vi "calculator.vi"() -> ()   [LabVIEW 2025]
uses:
  <vilib>/ErrorRing/Error Ring.xnode
panel:
  out "Run Time":string
  out "History":string[](array[string])
  out "result":dbl
  out "result str":string
  out "`()` count":u16
  in  "1/x":bool
  out "input queue":cluster{"op":u16, "number":dbl}[](array[cluster])
  in  "Stop":bool
  out "Current Time":string
  in  "C":bool
  in  "CE":bool
  in  "backspace":bool
  in  "sqrt":bool
  in  "+/-":bool
  in  "/":bool
  in  "=":bool
  in  "*":bool
  in  "-":bool
  in  "+":bool
  in  ".":bool
  in  "0":bool
  in  ")":bool
  in  "(":bool
  in  "9":bool
  in  "8":bool
  in  "7":bool
  in  "6":bool
  in  "5":bool
  in  "4":bool
  in  "3":bool
  in  "2":bool
  in  "1":bool
  out "screen":string
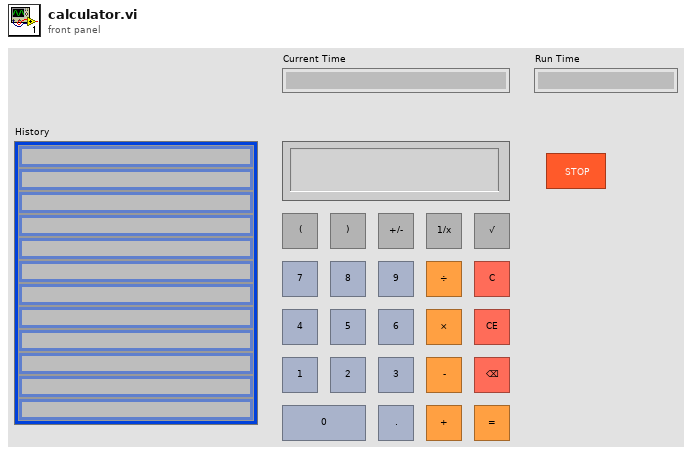
[diagram p1: front panel]
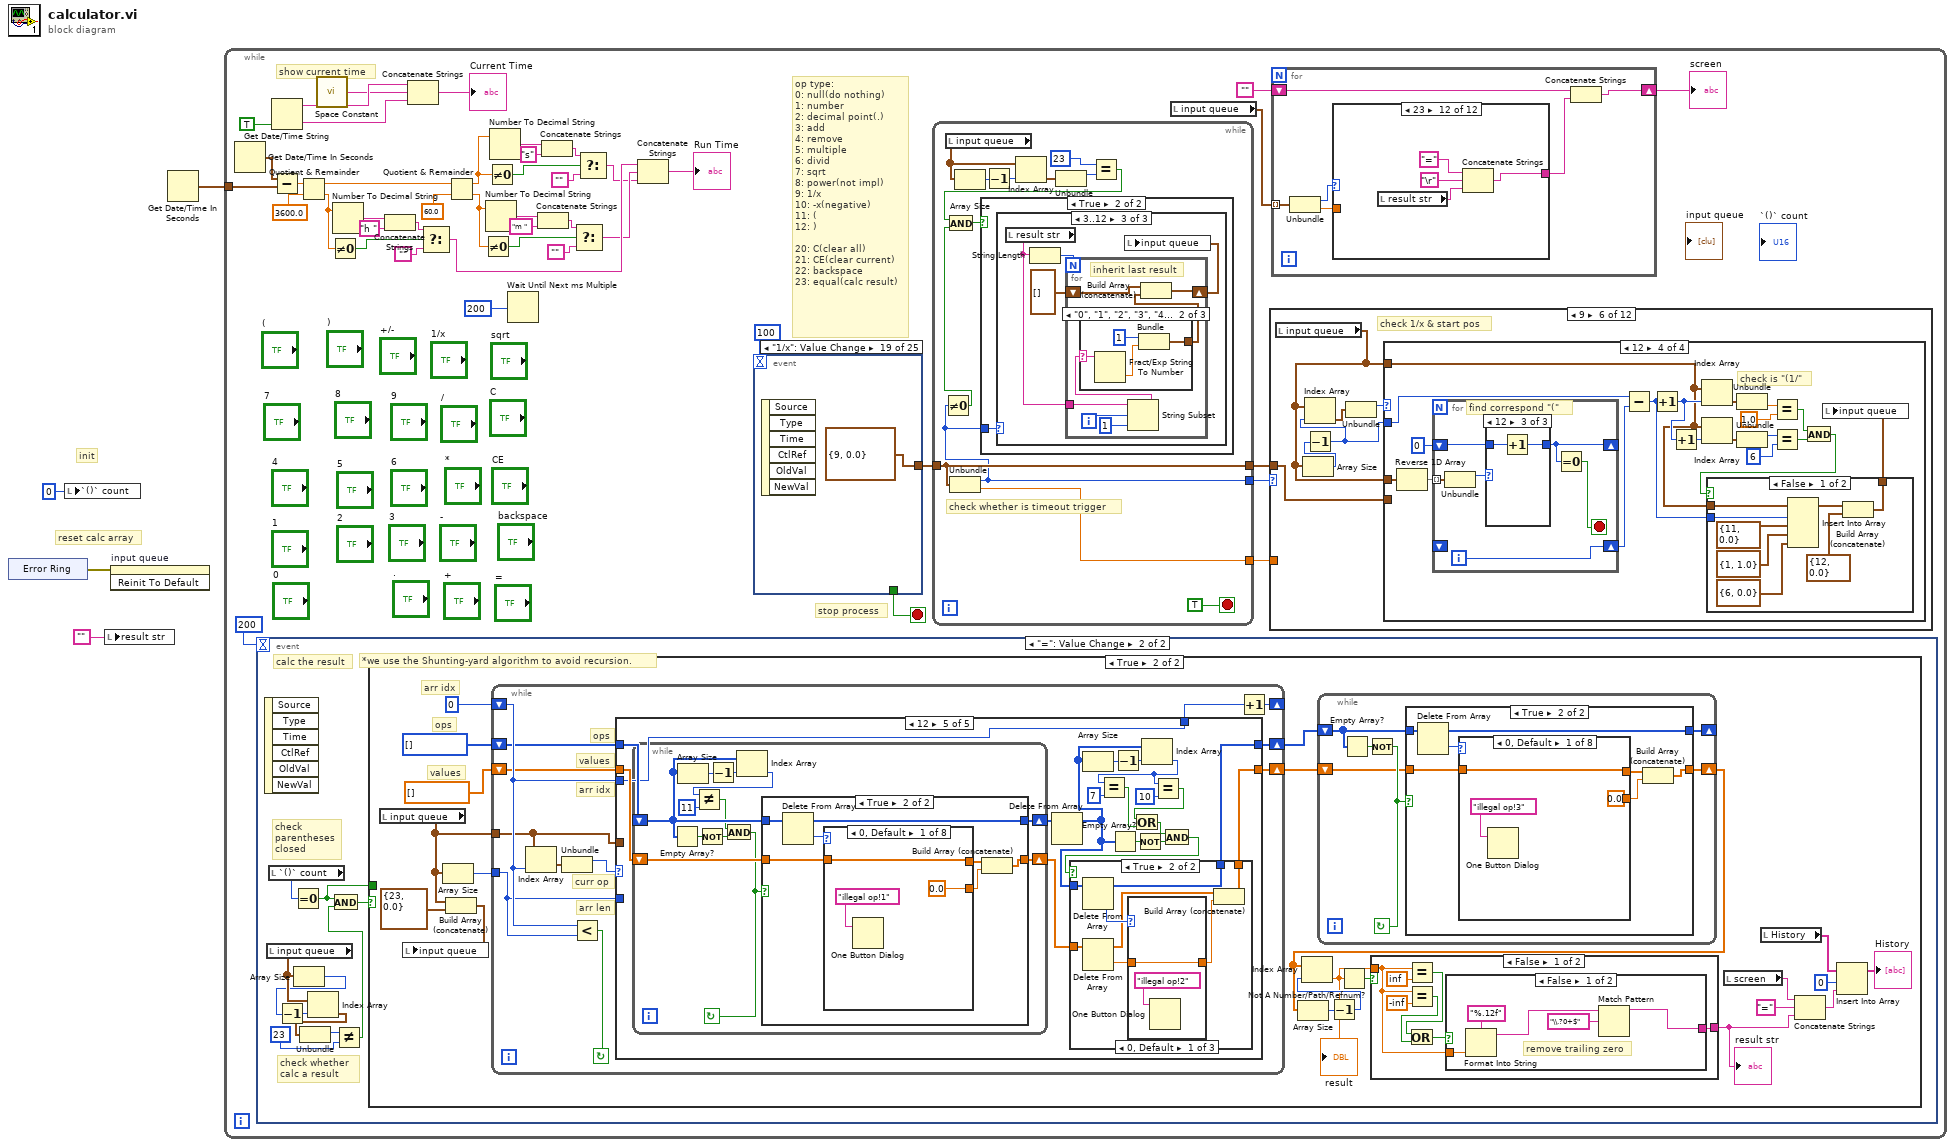
[diagram p0: block diagram]
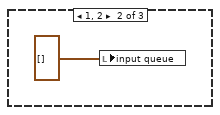
[diagram p4: hidden frame]
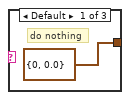
[diagram p5: hidden frame]
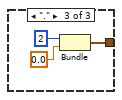
[diagram p6: hidden frame]
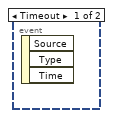
[diagram p7: hidden frame]
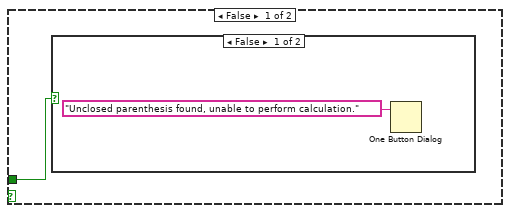
[diagram p8: hidden frame]
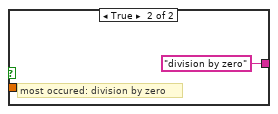
[diagram p10: hidden frame]
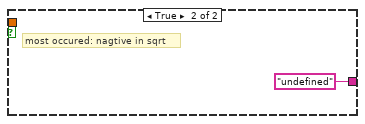
[diagram p11: hidden frame]
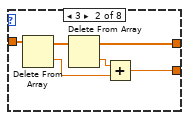
[diagram p13: hidden frame]
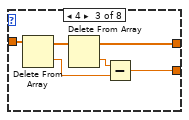
[diagram p14: hidden frame]
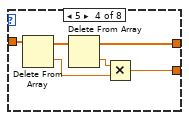
[diagram p15: hidden frame]
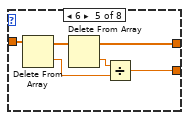
[diagram p16: hidden frame]
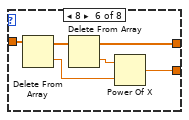
[diagram p17: hidden frame]
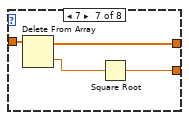
[diagram p18: hidden frame]
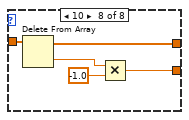
[diagram p19: hidden frame]
diagram:
  # "init"
  # "reset calc array"
  n1 = xnode "Error Ring"() -> ("error out"=w4:errorcluster)
  n2 = local write "`()` count"(u16 0 ("`()` count")) -> ()
  n3 = local write "result str"("" ("result str")) -> ()
  n4 = invoke on="input queue" class="Arr (strict)" method="Reinit To Default"(error in=w4) -> ()  [unwired: 2 in, 3 out]
  n5 = Get Date/Time In Seconds() -> (seconds since 1Jan1904=w1:timestamp)
  n6 = while {
    tunnel: w1 -> [w32]
    stop <- w37 stop-if-true
    # "stop process"
    # "op type:\n0: null(do nothing)\n1: number\n2: decimal point(.)\n3: add\n4: remove\n5: multiple\n6: divid\n7: sqrt\n8: power(not impl)\n9: 1/x\n10: -x(negative)\n11: (\n12: )\n\n20: C(clear all)\n21: CE(clear current)\n22: backspace\n23: equal(calc result)"
    # "show current time"
    n7 = Get Date/Time In Seconds() -> (seconds since 1Jan1904=w31:timestamp)
    n8 = event shown="[1] \"=\": Value Change" {
      selector: _ -> [_ _]
      dyn-events: _ -> [_ _]
      timeout: 200 -> [_ _]
      event Timeout {
        n9 = event-data() -> ()  [unwired: 1 in, 3 out]
      }
      event "=": Value Change {
        # "check whether\ncalc a result"
        # "check\nparentheses\nclosed"
        # "*we use the Shunting-yard algorithm to avoid recursion."
        # "calc the result"
        n10 = event-data() -> ()  [unwired: 1 in, 6 out]
        n11 = local read "input queue"() -> (w89:cluster{"op":u16, "number":dbl}[])
        n12 = local read "`()` count"() -> (w92:u16)
        n13 = Equal To 0?(x=w92) -> (x = 0?=w83:bool)
        n14 = Array Size(array=w89) -> (size(s)=w87:i32)
        n15 = Decrement(x=w87) -> (x-1=w88:i32)
        n16 = Index Array(array=w89, index=w88) -> (element=w90:cluster{"op":u16, "number":dbl})
        n17 = Unbundle(w90) -> ("op"=w91:u16)  [unwired: 1 out]
        n18 = Not Equal?(x=w91, y=u16 23) -> (x != y?=w85:bool)
        n19 = And(x=w83, y=w85) -> (x .and. y?=w84:bool)
        n20 = case shown="True" w84 {
          tunnel: w83 -> [w93 _]
          frame False {
            n21 = case shown="False" w93 {
              frame False {
                n22 = One Button Dialog(message="Unclosed parenthesis found, unable to perform calculation.") -> ()  [unwired: 1 in, 1 out]
              }
              frame True {
              }
            }
          }
          frame True {
            # "arr idx"
            # "ops"
            # "values"
            n23 = local read "input queue"() -> (w97:cluster{"op":u16, "number":dbl}[])
            n24 = Array Size(array=w97) -> (size(s)=w98:i32)
            n25 = Build Array (concatenate)(w97, cluster{u16, dbl} {23, 0.0}) -> (w96:cluster{"op":u16, "number":dbl}[])
            n26 = local write "input queue"(w96) -> ()
            n27 = while {
              shift-right: [w187] -> w111
              shift-left: dbl[] [] -> [w192]
              shift-right: [w194] -> w112
              shift-left: u16[] [] -> [w193]
              shift-right: [w190] -> _
              shift-left: 0 -> [w195]
              tunnel: w98 -> [w188]
              tunnel: w97 -> [w189]
              stop <- w198 continue-if-true
              # "values"
              # "ops"
              # "arr idx"
              # "arr len"
              # "curr op"
              n28 = Index Array(array=w189, index=w195) -> (element=w197:cluster{"op":u16, "number":dbl})
              n29 = Unbundle(w197) -> ("op"=w196:u16)  [unwired: 1 out]
              n30 = Less?(x=w195, y=w188) -> (x < y?=w198:bool)
              n31 = case shown="12" w196 {
                selector: w196 -> [_ _ w255 w317 _]
                tunnel: w195 -> [_ w215 w256 w319 w330]
                tunnel: [w200 w214 w256 w319 w330] -> w191
                tunnel: w188 -> [w200 w213 _ _ _]
                tunnel: [w201 w204 w254 w316 w320] -> w194
                tunnel: w193 -> [w201 w203 w253 w318 w338]
                tunnel: [w199 w209 w250 w315 w321] -> w187
                tunnel: w192 -> [w199 w210 w252 w315 w337]
                tunnel: w189 -> [_ w212 _ _ _]
                frame 0, Default {
                }
                frame 1 {
                  n32 = while {
                    shift-right: [w230] -> w211
                    shift-left: "" -> [w231]
                    shift-right: [w224] -> w214
                    shift-left: w215 -> [w225]
                    tunnel: w213 -> [w236]
                    tunnel: w212 -> [w235]
                    stop <- w226 continue-if-true
                    n33 = Index Array(array=w235, index=w225) -> (element=w234:cluster{"op":u16, "number":dbl})
                    n34 = Unbundle(w234) -> ("op"=w233:u16, "number"=w232:dbl)
                    n35 = Less?(x=w225, y=w236) -> (x < y?=w228:bool)
                    n36 = case shown="2" w233 {
                      tunnel: w232 -> [_ w245 _]
                      tunnel: ["" w244 "."] -> w229
                      tunnel: [FALSE TRUE TRUE] -> w227
                      tunnel: w225 -> [w238 w242 w246]
                      tunnel: [w237 w241 w247] -> w224
                      frame 0, Default {
                        n37 = Decrement(x=w238) -> (x-1=w237:i32)
                      }
                      frame 1 {
                        n38 = Number To Decimal String(number=w245) -> (decimal integer string=w244:string)  [unwired: 1 in]
                        n39 = Increment(x=w242) -> (x+1=w241:i32)
                      }
                      frame 2 {
                        n40 = Increment(x=w246) -> (x+1=w247:i32)
                      }
                    }
                    n41 = And(x=w227, y=w228) -> (x .and. y?=w226:bool)
                    n42 = Concatenate Strings(w231, w229) -> (w230:string)
                  }
                  n43 = Fract/Exp String To Number(string=w211) -> (number=w206:dbl)  [unwired: 3 in, 1 out]
                  n44 = Array Size(array=w203) -> (size(s)=w208:i32)
                  n45 = Decrement(x=w208) -> (x-1=w202:i32)
                  n46 = Index Array(array=w203, index=w202) -> (element=w207:u16)
                  n47 = case shown="10" w207 {
                    tunnel: w206 -> [w218 w223]
                    tunnel: [w218 w221] -> w205
                    tunnel: w203 -> [w217 w220]
                    tunnel: [w217 w219] -> w204
                    frame 0, Default {
                    }
                    frame 10 {
                      n48 = Delete From Array(array=w220) -> (array with subset deleted=w219:u16[])  [unwired: 2 in, 1 out]
                      n49 = Multiply(x=w223, y=-1.0) -> (x*y=w221:dbl)
                    }
                  }
                  n50 = Build Array (concatenate)(w210, w205) -> (w209:dbl[])
                }
                frame 3..6 {
                  n51 = while {
                    tunnel: w255 -> [w264]
                    shift-right: [w257] -> w250
                    shift-left: w252 -> [w259]
                    shift-right: [w258] -> w251
                    shift-left: w253 -> [w260]
                    stop <- w261 continue-if-true
                    n52 = case shown="3, 4" w264 {
                      tunnel: [i16 0 i16 1 i16 2 i16 3] -> w263
                      frame 0, Default {
                      }
                      frame 3, 4 {
                      }
                      frame 5, 6 {
                      }
                      frame 7 {
                      }
                    }
                    n53 = Empty Array?(array=w260) -> (empty?=w277:bool)
                    n54 = Array Size(array=w260) -> (size(s)=w275:i32)
                    n55 = Decrement(x=w275) -> (x-1=w274:i32)
                    n56 = Not(x=w277) -> (.not. x?=w276:bool)
                    n57 = Index Array(array=w260, index=w274) -> (element=w266:u16)
                    n58 = Not Equal?(x=w266, y=u16 7) -> (x != y?=w269:bool)
                    n59 = Not Equal?(x=w266, y=u16 11) -> (x != y?=w267:bool)
                    n60 = Not Equal?(x=w266, y=u16 12) -> (x != y?=w268:bool)
                    n61 = case shown="3, 4" w266 {
                      tunnel: [i16 0 i16 1 i16 2 i16 3] -> w265
                      frame 0, Default {
                      }
                      frame 3, 4 {
                      }
                      frame 5, 6 {
                      }
                      frame 7 {
                      }
                    }
                    n62 = Compound Arithmetic op=AND(w269, w267, w268) -> (w270:bool)
                    n63 = Greater Or Equal?(x=w265, y=w263) -> (x >= y?=w262:bool)
                    n64 = Compound Arithmetic op=AND(w276, w270, w262) -> (w261:bool)
                    n65 = case shown="True" w261 {
                      tunnel: w260 -> [w278 w289]
                      tunnel: w259 -> [w279 w288]
                      tunnel: [w279 w281] -> w257
                      tunnel: [w278 w280] -> w258
                      frame False {
                      }
                      frame True {
                        n66 = Delete From Array(array=w288) -> (deleted portion=w284:dbl, array with subset deleted=w286:dbl[])  [unwired: 2 in]
                        n67 = Delete From Array(array=w289) -> (deleted portion=w287:u16, array with subset deleted=w280:u16[])  [unwired: 2 in]
                        n68 = Delete From Array(array=w286) -> (deleted portion=w285:dbl, array with subset deleted=w283:dbl[])  [unwired: 2 in]
                        n69 = case shown="0, Default" w287 {
                          tunnel: w285 -> [w290 w294 w297 w300 w303 w306]
                          tunnel: w284 -> [_ w293 w296 w299 w302 w305]
                          tunnel: [w290 w292 w295 w298 w301 w304] -> w282
                          frame 0, Default {
                            n70 = One Button Dialog(message="illegal op!") -> ()  [unwired: 1 in, 1 out]
                          }
                          frame 3 {
                            n71 = Add(x=w294, y=w293) -> (x+y=w292:dbl)
                          }
                          frame 4 {
                            n72 = Subtract(x=w297, y=w296) -> (x-y=w295:dbl)
                          }
                          frame 5 {
                            n73 = Multiply(x=w300, y=w299) -> (x*y=w298:dbl)
                          }
                          frame 6 {
                            n74 = Divide(x=w303, y=w302) -> (x/y=w301:dbl)
                          }
                          frame 8 {
                            n75 = Power Of X(1:w305, 2:w306) -> (0:w304:dbl)
                          }
                        }
                        n76 = Build Array (concatenate)(w283, w282) -> (w281:dbl[])
                      }
                    }
                  }
                  n77 = Build Array (concatenate)(w251, w255) -> (w254:u16[])
                }
                frame 7, 8, 10, 11 {
                  n78 = Build Array (concatenate)(w318, w317) -> (w316:u16[])
                }
                frame 12 {
                  n79 = while {
                    shift-right: [w364] -> w336
                    shift-left: w338 -> [w361]
                    shift-right: [w365] -> w322
                    shift-left: w337 -> [w366]
                    stop <- w357 continue-if-true
                    n80 = Empty Array?(array=w361) -> (empty?=w367:bool)
                    n81 = Array Size(array=w361) -> (size(s)=w363:i32)
                    n82 = Not(x=w367) -> (.not. x?=w358:bool)
                    n83 = Decrement(x=w363) -> (x-1=w362:i32)
                    n84 = Index Array(array=w361, index=w362) -> (element=w360:u16)
                    n85 = Not Equal?(x=w360, y=u16 11) -> (x != y?=w356:bool)
                    n86 = And(x=w356, y=w358) -> (x .and. y?=w357:bool)
                    n87 = case shown="True" w357 {
                      tunnel: [w369 w375] -> w365
                      tunnel: w361 -> [w368 w374]
                      tunnel: w366 -> [w369 w372]
                      tunnel: [w368 w370] -> w364
                      frame False {
                      }
                      frame True {
                        n88 = Delete From Array(array=w374) -> (deleted portion=w373:u16, array with subset deleted=w370:u16[])  [unwired: 2 in]
                        n89 = case shown="0, Default" w373 {
                          tunnel: [0.0 w385 w391 w397 w403 w409 w413 w418] -> w376
                          tunnel: w372 -> [w378 w384 w390 w396 w402 w408 w412 w417]
                          tunnel: [w378 w382 w388 w394 w400 w406 w410 w416] -> w371
                          frame 0, Default {
                            n90 = One Button Dialog(message="illegal op!1") -> ()  [unwired: 1 in, 1 out]
                          }
                          frame 3 {
                            n91 = Delete From Array(array=w384) -> (deleted portion=w380:dbl, array with subset deleted=w383:dbl[])  [unwired: 2 in]
                            n92 = Delete From Array(array=w383) -> (deleted portion=w381:dbl, array with subset deleted=w382:dbl[])  [unwired: 2 in]
                            n93 = Add(x=w381, y=w380) -> (x+y=w385:dbl)
                          }
                          frame 4 {
                            n94 = Delete From Array(array=w390) -> (deleted portion=w386:dbl, array with subset deleted=w389:dbl[])  [unwired: 2 in]
                            n95 = Delete From Array(array=w389) -> (deleted portion=w387:dbl, array with subset deleted=w388:dbl[])  [unwired: 2 in]
                            n96 = Subtract(x=w387, y=w386) -> (x-y=w391:dbl)
                          }
                          frame 5 {
                            n97 = Delete From Array(array=w396) -> (deleted portion=w392:dbl, array with subset deleted=w395:dbl[])  [unwired: 2 in]
                            n98 = Delete From Array(array=w395) -> (deleted portion=w393:dbl, array with subset deleted=w394:dbl[])  [unwired: 2 in]
                            n99 = Multiply(x=w393, y=w392) -> (x*y=w397:dbl)
                          }
                          frame 6 {
                            n100 = Delete From Array(array=w402) -> (deleted portion=w398:dbl, array with subset deleted=w401:dbl[])  [unwired: 2 in]
                            n101 = Delete From Array(array=w401) -> (deleted portion=w399:dbl, array with subset deleted=w400:dbl[])  [unwired: 2 in]
                            n102 = Divide(x=w399, y=w398) -> (x/y=w403:dbl)
                          }
                          frame 8 {
                            n103 = Delete From Array(array=w408) -> (deleted portion=w404:dbl, array with subset deleted=w407:dbl[])  [unwired: 2 in]
                            n104 = Delete From Array(array=w407) -> (deleted portion=w405:dbl, array with subset deleted=w406:dbl[])  [unwired: 2 in]
                            n105 = Power Of X(1:w404, 2:w405) -> (0:w409:dbl)
                          }
                          frame 7 {
                            n106 = Delete From Array(array=w412) -> (deleted portion=w411:dbl, array with subset deleted=w410:dbl[])  [unwired: 2 in]
                            n107 = Square Root(x=w411) -> (sqrt(x)=w413:dbl)
                          }
                          frame 10 {
                            n108 = Delete From Array(array=w417) -> (deleted portion=w415:dbl, array with subset deleted=w416:dbl[])  [unwired: 2 in]
                            n109 = Multiply(x=w415, y=-1.0) -> (x*y=w418:dbl)
                          }
                        }
                        n110 = Build Array (concatenate)(w371, w376) -> (w375:dbl[])
                      }
                    }
                  }
                  n111 = Delete From Array(array=w336) -> (array with subset deleted=w323:u16[])  [unwired: 2 in, 1 out]
                  n112 = Array Size(array=w323) -> (size(s)=w332:i32)
                  n113 = Empty Array?(array=w323) -> (empty?=w331:bool)
                  n114 = Decrement(x=w332) -> (x-1=w333:i32)
                  n115 = Not(x=w331) -> (.not. x?=w335:bool)
                  n116 = Index Array(array=w323, index=w333) -> (element=w328:u16)
                  n117 = Equal?(x=w328, y=u16 7) -> (x = y?=w326:bool)
                  n118 = Equal?(x=w328, y=u16 10) -> (x = y?=w325:bool)
                  n119 = Or(x=w325, y=w326) -> (x .or. y?=w327:bool)
                  n120 = And(x=w327, y=w335) -> (x .and. y?=w324:bool)
                  n121 = case shown="True" w324 {
                    tunnel: w323 -> [w340 w348]
                    tunnel: w322 -> [w339 w347]
                    tunnel: [w339 w344] -> w321
                    tunnel: [w340 w341] -> w320
                    frame False {
                    }
                    frame True {
                      n122 = Delete From Array(array=w348) -> (deleted portion=w346:u16, array with subset deleted=w341:u16[])  [unwired: 2 in]
                      n123 = Delete From Array(array=w347) -> (deleted portion=w345:dbl, array with subset deleted=w343:dbl[])  [unwired: 2 in]
                      n124 = case shown="0, Default" w346 {
                        tunnel: w345 -> [w350 w352 w355]
                        tunnel: [w350 w351 w353] -> w342
                        frame 0, Default {
                          n125 = One Button Dialog(message="illegal op!2") -> ()  [unwired: 1 in, 1 out]
                        }
                        frame 7 {
                          n126 = Square Root(x=w352) -> (sqrt(x)=w351:dbl)
                        }
                        frame 10 {
                          n127 = Multiply(x=w355, y=-1.0) -> (x*y=w353:dbl)
                        }
                      }
                      n128 = Build Array (concatenate)(w343, w342) -> (w344:dbl[])
                    }
                  }
                }
              }
              n129 = Increment(x=w191) -> (x+1=w190:i32)
            }
            n130 = while {
              shift-right: [w130] -> _
              shift-left: w112 -> [w133]
              shift-right: [w131] -> w107
              shift-left: w111 -> [w132]
              stop <- w134 continue-if-true
              n131 = Empty Array?(array=w133) -> (empty?=w135:bool)
              n132 = Not(x=w135) -> (.not. x?=w134:bool)
              n133 = case shown="True" w134 {
                tunnel: [w137 w143] -> w131
                tunnel: w133 -> [w136 w142]
                tunnel: w132 -> [w137 w140]
                tunnel: [w136 w138] -> w130
                frame False {
                }
                frame True {
                  n134 = Delete From Array(array=w142) -> (deleted portion=w141:u16, array with subset deleted=w138:u16[])  [unwired: 2 in]
                  n135 = case shown="0, Default" w141 {
                    tunnel: [0.0 w153 w159 w165 w171 w177 w181 w186] -> w144
                    tunnel: w140 -> [w146 w152 w158 w164 w170 w176 w180 w185]
                    tunnel: [w146 w150 w156 w162 w168 w174 w178 w184] -> w139
                    frame 0, Default {
                      n136 = One Button Dialog(message="illegal op!3") -> ()  [unwired: 1 in, 1 out]
                    }
                    frame 3 {
                      n137 = Delete From Array(array=w152) -> (deleted portion=w148:dbl, array with subset deleted=w151:dbl[])  [unwired: 2 in]
                      n138 = Delete From Array(array=w151) -> (deleted portion=w149:dbl, array with subset deleted=w150:dbl[])  [unwired: 2 in]
                      n139 = Add(x=w149, y=w148) -> (x+y=w153:dbl)
                    }
                    frame 4 {
                      n140 = Delete From Array(array=w158) -> (deleted portion=w154:dbl, array with subset deleted=w157:dbl[])  [unwired: 2 in]
                      n141 = Delete From Array(array=w157) -> (deleted portion=w155:dbl, array with subset deleted=w156:dbl[])  [unwired: 2 in]
                      n142 = Subtract(x=w155, y=w154) -> (x-y=w159:dbl)
                    }
                    frame 5 {
                      n143 = Delete From Array(array=w164) -> (deleted portion=w160:dbl, array with subset deleted=w163:dbl[])  [unwired: 2 in]
                      n144 = Delete From Array(array=w163) -> (deleted portion=w161:dbl, array with subset deleted=w162:dbl[])  [unwired: 2 in]
                      n145 = Multiply(x=w161, y=w160) -> (x*y=w165:dbl)
                    }
                    frame 6 {
                      n146 = Delete From Array(array=w170) -> (deleted portion=w166:dbl, array with subset deleted=w169:dbl[])  [unwired: 2 in]
                      n147 = Delete From Array(array=w169) -> (deleted portion=w167:dbl, array with subset deleted=w168:dbl[])  [unwired: 2 in]
                      n148 = Divide(x=w167, y=w166) -> (x/y=w171:dbl)
                    }
                    frame 8 {
                      n149 = Delete From Array(array=w176) -> (deleted portion=w172:dbl, array with subset deleted=w175:dbl[])  [unwired: 2 in]
                      n150 = Delete From Array(array=w175) -> (deleted portion=w173:dbl, array with subset deleted=w174:dbl[])  [unwired: 2 in]
                      n151 = Power Of X(1:w172, 2:w173) -> (0:w177:dbl)
                    }
                    frame 7 {
                      n152 = Delete From Array(array=w180) -> (deleted portion=w179:dbl, array with subset deleted=w178:dbl[])  [unwired: 2 in]
                      n153 = Square Root(x=w179) -> (sqrt(x)=w181:dbl)
                    }
                    frame 10 {
                      n154 = Delete From Array(array=w185) -> (deleted portion=w183:dbl, array with subset deleted=w184:dbl[])  [unwired: 2 in]
                      n155 = Multiply(x=w183, y=-1.0) -> (x*y=w186:dbl)
                    }
                  }
                  n156 = Build Array (concatenate)(w139, w144) -> (w143:dbl[])
                }
              }
            }
            n157 = Array Size(array=w107) -> (size(s)=w110:i32)
            n158 = Decrement(x=w110) -> (x-1=w109:i32)
            n159 = Index Array(array=w107, index=w109) -> (element=w106:dbl)
            "result" <- w106
            n160 = Not A Number/Path/Refnum?(number/path/refnum=w106) -> (NaN/Path/Refnum?=w108:bool)
            n161 = case shown="False" w108 {
              tunnel: w106 -> [w116 _]
              tunnel: [w117 "undefined" ("result")] -> w99
              frame False {
                n162 = Equal?(x=w116, y=inf) -> (x = y?=w119:bool)
                n163 = Equal?(x=w116, y=-inf) -> (x = y?=w120:bool)
                n164 = Or(x=w119, y=w120) -> (x .or. y?=w118:bool)
                n165 = case shown="False" w118 {
                  tunnel: [w123 "division by zero"] -> w117
                  tunnel: w116 -> [w127 _]
                  frame False {
                    # "remove trailing zero"
                    n166 = Format Into String(format string="%.12f", w127) -> (resulting string=w125:string)  [unwired: 2 in, 1 out]
                    n167 = Match Pattern(string=w125, regular expression="\\.?0+$") -> (before substring=w123:string)  [unwired: 1 in, 3 out]
                  }
                  frame True {
                    # "most occured: division by zero"
                  }
                }
              }
              frame True {
                # "most occured: nagtive in sqrt"
              }
            }
            "result str" <- w99
            n168 = local read "screen"() -> (w105:string)
            n169 = local read "History"() -> (w103:string[])
            n170 = Concatenate Strings(w105, "=" ("string"), w99) -> (w102:string)
            n171 = Insert Into Array(array=w103, index=0, new element=w102) -> (→"History":string[])
          }
        }
      }
    }
    n172 = Get Date/Time String(want seconds? (F)=TRUE) -> (date string=w46:string, time string=w45:string)  [unwired: 2 in]
    n173 = Subtract(x=w31, y=w32) -> (x-y=w30:dbl)
    n174 = Quotient & Remainder(x=w30, y=3600.0) -> (x-y*floor(x/y)=w28:dbl, floor(x/y)=w25:dbl)
    n175 = call <vilib>:"Space Constant.vi"() -> ("String"=w44:string)
    n176 = Not Equal To 0?(x=w25) -> (x != 0?=w26:bool)
    n177 = Number To Decimal String(number=w25) -> (decimal integer string=w24:string)  [unwired: 1 in]
    n178 = Concatenate Strings(w24, "h " ("string")) -> (w22:string)
    n179 = Concatenate Strings(w46, w44, w45) -> (→"Current Time":string)
    n180 = Select(t=w22, s=w26, f="") -> (s? t:f=w8:string)
    n181 = Quotient & Remainder(x=w28, y=60.0) -> (x-y*floor(x/y)=w9:dbl, floor(x/y)=w16:dbl)
    n182 = Not Equal To 0?(x=w16) -> (x != 0?=w17:bool)
    n183 = Number To Decimal String(number=w16) -> (decimal integer string=w15:string)  [unwired: 1 in]
    n184 = Not Equal To 0?(x=w9) -> (x != 0?=w13:bool)
    n185 = Number To Decimal String(number=w9) -> (decimal integer string=w14:string)  [unwired: 1 in]
    n186 = Wait Until Next ms Multiple(millisecond multiple=200) -> ()  [unwired: 1 out]
    n187 = Concatenate Strings(w15, "m " ("string")) -> (w19:string)
    n188 = Concatenate Strings(w14, "s" ("string")) -> (w11:string)
    n189 = Select(t=w19, s=w17, f="") -> (s? t:f=w7:string)
    n190 = Select(t=w11, s=w13, f="") -> (s? t:f=w6:string)
    n191 = Concatenate Strings(w8, w7, w6) -> (→"Run Time":string)
    n192 = event shown="[18] \"1/x\": Value Change" {
      selector: _ -> [_ _ _ _ _ _ _ _ _ _ _ _ _ _ _ _ _ _ _ _ _ _ _ _ _]
      dyn-events: _ -> [_ _ _ _ _ _ _ _ _ _ _ _ _ _ _ _ _ _ _ _ _ _ _ _ _]
      timeout: 100 -> [_ _ _ _ _ _ _ _ _ _ _ _ _ _ _ _ _ _ _ _ _ _ _ _ _]
      tunnel: [_ _ cluster{u16, dbl} {1, 1.0} cluster{u16, dbl} {1, 2.0} cluster{u16, dbl} {1, 3.0} cluster{u16, dbl} {1, 4.0} cluster{u16, dbl} {1, 5.0} cluster{u16, dbl} {1, 6.0} cluster{u16, dbl} {1, 7.0} cluster{u16, dbl} {1, 8.0} cluster{u16, dbl} {1, 9.0} cluster{u16, dbl} {1, 0.0} cluster{u16, dbl} {2, 0.0} cluster{u16, dbl} {3, 0.0} cluster{u16, dbl} {4, 0.0} cluster{u16, dbl} {5, 0.0} cluster{u16, dbl} {6, 0.0} cluster{u16, dbl} {7, 0.0} cluster{u16, dbl} {9, 0.0} cluster{u16, dbl} {10, 0.0} cluster{u16, dbl} {11, 0.0} cluster{u16, dbl} {12, 0.0} cluster{u16, dbl} {20, 0.0} cluster{u16, dbl} {21, 0.0} cluster{u16, dbl} {22, 0.0}] -> w34
      tunnel: [_ "Stop" _ _ _ _ _ _ _ _ _ _ _ _ _ _ _ _ _ _ _ _ _ _ _] -> w37
      event Timeout {
        n193 = event-data() -> ()  [unwired: 1 in, 3 out]
      }
      event "Stop": Value Change {
        n194 = event-data() -> ()  [unwired: 1 in, 6 out]
      }
      event "1": Value Change {
        n195 = event-data() -> ()  [unwired: 1 in, 6 out]
      }
      event "2": Value Change {
        n196 = event-data() -> ()  [unwired: 1 in, 6 out]
      }
      event "3": Value Change {
        n197 = event-data() -> ()  [unwired: 1 in, 6 out]
      }
      event "4": Value Change {
        n198 = event-data() -> ()  [unwired: 1 in, 6 out]
      }
      event "5": Value Change {
        n199 = event-data() -> ()  [unwired: 1 in, 6 out]
      }
      event "6": Value Change {
        n200 = event-data() -> ()  [unwired: 1 in, 6 out]
      }
      event "7": Value Change {
        n201 = event-data() -> ()  [unwired: 1 in, 6 out]
      }
      event "8": Value Change {
        n202 = event-data() -> ()  [unwired: 1 in, 6 out]
      }
      event "9": Value Change {
        n203 = event-data() -> ()  [unwired: 1 in, 6 out]
      }
      event "0": Value Change {
        n204 = event-data() -> ()  [unwired: 1 in, 6 out]
      }
      event ".": Value Change {
        n205 = event-data() -> ()  [unwired: 1 in, 6 out]
      }
      event "+": Value Change {
        n206 = event-data() -> ()  [unwired: 1 in, 6 out]
      }
      event "-": Value Change {
        n207 = event-data() -> ()  [unwired: 1 in, 6 out]
      }
      event "*": Value Change {
        n208 = event-data() -> ()  [unwired: 1 in, 6 out]
      }
      event "/": Value Change {
        n209 = event-data() -> ()  [unwired: 1 in, 6 out]
      }
      event "sqrt": Value Change {
        n210 = event-data() -> ()  [unwired: 1 in, 6 out]
      }
      event "1/x": Value Change {
        n211 = event-data() -> ()  [unwired: 1 in, 6 out]
      }
      event "+/-": Value Change {
        n212 = event-data() -> ()  [unwired: 1 in, 6 out]
      }
      event "(": Value Change {
        n213 = event-data() -> ()  [unwired: 1 in, 6 out]
      }
      event ")": Value Change {
        n214 = event-data() -> ()  [unwired: 1 in, 6 out]
      }
      event "C": Value Change {
        n215 = event-data() -> ()  [unwired: 1 in, 6 out]
      }
      event "CE": Value Change {
        n216 = event-data() -> ()  [unwired: 1 in, 6 out]
      }
      event "backspace": Value Change {
        n217 = event-data() -> ()  [unwired: 1 in, 6 out]
      }
    }
    n218 = while {
      tunnel: [w54] -> w33
      tunnel: w34 -> [w54]
      tunnel: [w49] -> w36
      tunnel: [w53] -> w35
      stop <- TRUE stop-if-true
      # "check whether is timeout trigger"
      n219 = local read "input queue"() -> (w59:cluster{"op":u16, "number":dbl}[])
      n220 = Unbundle(w54) -> (w49:u16, w53:dbl)
      n221 = Not Equal To 0?(x=w49) -> (x != 0?=w52:bool)
      n222 = Array Size(array=w59) -> (size(s)=w58:i32)
      n223 = Decrement(x=w58) -> (x-1=w57:i32)
      n224 = Index Array(array=w59, index=w57) -> (element=w60:cluster{"op":u16, "number":dbl})
      n225 = Unbundle(w60) -> ("op"=w56:u16)  [unwired: 1 out]
      n226 = Equal?(x=u16 23, y=w56) -> (x = y?=w50:bool)
      n227 = And(x=w50, y=w52) -> (x .and. y?=w51:bool)
      n228 = case shown="True" w51 {
        tunnel: w49 -> [_ w62]
        frame False {
        }
        frame True {
          n229 = case shown="3..12" w62 {
            frame 0, Default {
            }
            frame 1, 2 {
              n230 = local write "input queue"(cluster{u16, dbl}[] []) -> ()
            }
            frame 3..12 {
              n231 = local read "result str"() -> (w67:string)
              n232 = String Length(string=w67) -> (length=w66:i32)
              n233 = for {
                N: w66 -> [_]
                shift-right: [w68] -> w65
                shift-left: cluster{u16, dbl}[] [] -> [w69]
                tunnel: w67 -> [w72]
                i -> [w73]
                # "inherit last result"
                n234 = String Subset(string=w72, offset (0)=w73, length (rest)=1 ("length (rest)")) -> (substring=w71:string)
                n235 = case shown="\"0\", \"1\", \"2\", \"3\", \"4\", \"5\", \"6\", \"7\", \"8\", \"9\"" w71 {
                  selector: w71 -> [_ w76 _]
                  tunnel: [cluster{u16, dbl} {0, 0.0} w77 w81] -> w70
                  frame Default {
                    # "do nothing"
                  }
                  frame "0", "1", "2", "3", "4", "5", "6", "7", "8", "9" {
                    n236 = Fract/Exp String To Number(string=w76) -> (number=w78:dbl)  [unwired: 3 in, 1 out]
                    n237 = Bundle(u16 1, w78) -> (w77:cluster{u16, dbl})  [unwired: 1 in]
                  }
                  frame "." {
                    n238 = Bundle(u16 2, 0.0) -> (w81:cluster{u16, dbl})  [unwired: 1 in]
                  }
                }
                n239 = Build Array (concatenate)(w69, w70) -> (w68:cluster{u16, dbl}[])
              }
              n240 = local write "input queue"(w65) -> ()
            }
          }
        }
      }
    }
    n241 = local read "input queue"() -> (w40:cluster{"op":u16, "number":dbl}[])
    n242 = case shown="9" w36 {
      tunnel: w33 -> [_ w443 w448 w474 w491 w529 w620 w685 w702 _ _ _]
      tunnel: w35 -> [_ _ _ _ _ _ _ _ _ _ _ _]
      frame 0 {
        # "op = 0, do nothing"
      }
      frame 1, Default {
        n243 = local read "input queue"() -> (w441:cluster{"op":u16, "number":dbl}[])
        n244 = Build Array (concatenate)(w441, w443) -> (w442:cluster{"op":u16, "number":dbl}[])
        n245 = local write "input queue"(w442) -> ()
      }
      frame 2 {
        # "check dot"
        n246 = local read "input queue"() -> (w444:cluster{"op":u16, "number":dbl}[])
        n247 = Reverse 1D Array(array=w444) -> (reversed array=w447:cluster{"op":u16, "number":dbl}[])
        n248 = for {
          tunnel: w447 -> [w454] mode=indexing
          shift-right: [w449] -> w445
          shift-left: FALSE -> [_]
          stop <- w452 stop-if-true
          n249 = Unbundle(w454) -> ("op"=w451:u16)  [unwired: 1 out]
          n250 = Not Equal?(x=w451, y=u16 1) -> (x != y?=w452:bool)
          n251 = Equal?(x=u16 2, y=w451) -> (x = y?=w449:bool)
        }
        n252 = case shown="False" w445 {
          tunnel: w448 -> [w457 _]
          tunnel: w444 -> [w455 _]
          frame False {
            n253 = Array Size(array=w455) -> (size(s)=w463:i32)
            n254 = Decrement(x=w463) -> (x-1=w462:i32)
            n255 = Index Array(array=w455, index=w462) -> (element=w461:cluster{"op":u16, "number":dbl})
            n256 = Unbundle(w461) -> ("op"=w460:u16)  [unwired: 1 out]
            n257 = Not Equal?(x=w460, y=u16 1) -> (x != y?=w458:bool)
            n258 = case shown="True" w458 {
              tunnel: w455 -> [w466 w470]
              tunnel: w457 -> [w465 w469]
              tunnel: [w464 w467] -> w456
              frame False {
                n259 = Build Array (concatenate)(w466, w465) -> (w464:cluster{"op":u16, "number":dbl}[])
              }
              frame True {
                n260 = Build Array (concatenate)(w470, cluster{u16, dbl} {1, 0.0}, w469) -> (w467:cluster{"op":u16, "number":dbl}[])
              }
            }
            n261 = local write "input queue"(w456) -> ()
          }
          frame True {
            n262 = One Button Dialog(message="There's already a decimal point.") -> ()  [unwired: 1 in, 1 out]
          }
        }
      }
      frame 3..6 {
        # "can only put ops(+-*/) after number or \")\""
        n263 = local read "input queue"() -> (w475:cluster{"op":u16, "number":dbl}[])
        n264 = Array Size(array=w475) -> (size(s)=w477:i32)
        n265 = Decrement(x=w477) -> (x-1=w472:i32)
        n266 = Index Array(array=w475, index=w472) -> (element=w476:cluster{"op":u16, "number":dbl})
        n267 = Unbundle(w476) -> ("op"=w473:u16)  [unwired: 1 out]
        n268 = case shown="1, 12" w473 {
          tunnel: w475 -> [_ w480 w484]
          tunnel: w474 -> [_ w479 w483]
          tunnel: w472 -> [_ _ w482]
          frame 0, Default {
            n269 = One Button Dialog(message="You can't place operators here!") -> ()  [unwired: 1 in, 1 out]
          }
          frame 1, 12 {
            n270 = Build Array (concatenate)(w480, w479) -> (w481:cluster{"op":u16, "number":dbl}[])
            n271 = local write "input queue"(w481) -> ()
          }
          frame 3..6 {
            n272 = Replace Array Subset(array=w484, new element=w483, index=w482) -> (w485:cluster{"op":u16, "number":dbl}[])
            n273 = local write "input queue"(w485) -> ()
          }
        }
      }
      frame 7 {
        # "check sqrt & start pos"
        n274 = local read "input queue"() -> (w489:cluster{"op":u16, "number":dbl}[])
        n275 = Array Size(array=w489) -> (size(s)=w487:i32)
        n276 = Decrement(x=w487) -> (x-1=w486:i32)
        n277 = Index Array(array=w489, index=w486) -> (element=w490:cluster{"op":u16, "number":dbl})
        n278 = Unbundle(w490) -> ("op"=w488:u16)  [unwired: 1 out]
        n279 = case shown="1, 2" w488 {
          tunnel: w491 -> [w496 w498 _ w524]
          tunnel: w489 -> [w497 w505 _ w527]
          tunnel: w486 -> [_ w506 _ _]
          frame 0, 3..6, 11 {
            n280 = Build Array (concatenate)(w497, w496, cluster{u16, dbl} {11, 0.0}) -> (w494:cluster{"op":u16, "number":dbl}[])
            n281 = local write "input queue"(w494) -> ()
            n282 = local read "`()` count"() -> (w493:u16)
            n283 = Increment(x=w493) -> (x+1=w492:u16)
            n284 = local write "`()` count"(w492) -> ()
          }
          frame 1, 2 {
            n285 = Reverse 1D Array(array=w505) -> (reversed array=w507:cluster{"op":u16, "number":dbl}[])
            n286 = for {
              tunnel: w507 -> [w516] mode=indexing
              shift-right: [w513] -> w499
              shift-left: _ -> [_]
              i -> [w514]
              stop <- w508 stop-if-true
              n287 = Unbundle(w516) -> ("op"=w511:u16)  [unwired: 1 out]
              n288 = Not Equal?(x=w511, y=u16 1) -> (x != y?=w510:bool)
              n289 = Not Equal?(x=w511, y=u16 2) -> (x != y?=w509:bool)
              n290 = And(x=w510, y=w509) -> (x .and. y?=w508:bool)
              n291 = case shown="True" w508 {
                tunnel: w514 -> [w517 w519]
                tunnel: [w517 w518] -> w513
                frame False {
                }
                frame True {
                  n292 = Decrement(x=w519) -> (x-1=w518:i32)
                }
              }
            }
            n293 = Subtract(x=w506, y=w499) -> (x-y=w504:i32)
            n294 = Insert Into Array(array=w505, index=w504, new element #1=w498, new element #2=cluster{u16, dbl} {11, 0.0}) -> (w500:cluster{"op":u16, "number":dbl}[])
            n295 = Build Array (concatenate)(w500, cluster{u16, dbl} {12, 0.0}) -> (w501:cluster{"op":u16, "number":dbl}[])
            n296 = local write "input queue"(w501) -> ()
          }
          frame 7, Default {
            n297 = One Button Dialog(message="You can't place sqrt here!") -> ()  [unwired: 1 in, 1 out]
          }
          frame 12 {
            n298 = Build Array (concatenate)(w527, cluster{u16, dbl} {5, 0.0}, w524, cluster{u16, dbl} {11, 0.0}) -> (w526:cluster{"op":u16, "number":dbl}[])
            n299 = local read "`()` count"() -> (w522:u16)
            n300 = local write "input queue"(w526) -> ()
            n301 = Increment(x=w522) -> (x+1=w521:u16)
            n302 = local write "`()` count"(w521) -> ()
          }
        }
      }
      frame 9 {
        # "check 1/x & start pos"
        n303 = local read "input queue"() -> (w528:cluster{"op":u16, "number":dbl}[])
        n304 = Array Size(array=w528) -> (size(s)=w531:i32)
        n305 = Decrement(x=w531) -> (x-1=w530:i32)
        n306 = Index Array(array=w528, index=w530) -> (element=w533:cluster{"op":u16, "number":dbl})
        n307 = Unbundle(w533) -> ("op"=w532:u16)  [unwired: 1 out]
        n308 = case shown="12" w532 {
          tunnel: w528 -> [_ w537 w576 w595]
          tunnel: w530 -> [_ w541 _ w592]
          tunnel: w529 -> [_ _ _ _]
          tunnel: w528 -> [_ _ _ w579]
          frame 7, Default {
            n309 = One Button Dialog(message="You can't place negative here!") -> ()  [unwired: 1 in, 1 out]
          }
          frame 1, 2 {
            n310 = Reverse 1D Array(array=w537) -> (reversed array=w542:cluster{"op":u16, "number":dbl}[])
            n311 = for {
              tunnel: w542 -> [w566] mode=indexing
              shift-right: [w564] -> w539
              shift-left: _ -> [_]
              i -> [w565]
              stop <- w558 stop-if-true
              n312 = Unbundle(w566) -> ("op"=w562:u16)  [unwired: 1 out]
              n313 = Not Equal?(x=w562, y=u16 1) -> (x != y?=w560:bool)
              n314 = Not Equal?(x=w562, y=u16 2) -> (x != y?=w559:bool)
              n315 = And(x=w560, y=w559) -> (x .and. y?=w558:bool)
              n316 = case shown="False" w558 {
                tunnel: w565 -> [w568 w569]
                tunnel: [w567 w569] -> w564
                frame False {
                  n317 = Increment(x=w568) -> (x+1=w567:i32)
                }
                frame True {
                }
              }
            }
            n318 = Subtract(x=w541, y=w539) -> (x-y=w538:i32)
            n319 = Index Array(array=w537, index=w538) -> (element=w536:cluster{"op":u16, "number":dbl})
            n320 = Unbundle(w536) -> ("op"=w535:u16)  [unwired: 1 out]
            n321 = case shown="3..6, Default" w535 {
              tunnel: [w548 w551] -> w540
              tunnel: w538 -> [_ w557]
              tunnel: w537 -> [w546 w556]
              frame 0 {
                n322 = Build Array (concatenate)(cluster{u16, dbl} {11, 0.0}, cluster{u16, dbl} {1, 1.0}, cluster{u16, dbl} {6, 0.0}, w546, cluster{u16, dbl} {12, 0.0}) -> (w548:cluster{"op":u16, "number":dbl}[])
              }
              frame 3..6, Default {
                n323 = Increment(x=w557) -> (x+1=w555:i32)
                n324 = Insert Into Array(array=w556, index=w555, new element #1=cluster{u16, dbl} {11, 0.0}, new element #2=cluster{u16, dbl} {1, 1.0}, new element #3=cluster{u16, dbl} {6, 0.0}) -> (w550:cluster{"op":u16, "number":dbl}[])
                n325 = Build Array (concatenate)(w550, cluster{u16, dbl} {12, 0.0}) -> (w551:cluster{"op":u16, "number":dbl}[])
              }
            }
            n326 = local write "input queue"(w540) -> ()
          }
          frame 0, 3..6, 11 {
            n327 = Build Array (concatenate)(w576, cluster{u16, dbl} {11, 0.0}, cluster{u16, dbl} {1, 1.0}, cluster{u16, dbl} {6, 0.0}) -> (w575:cluster{"op":u16, "number":dbl}[])
            n328 = local write "input queue"(w575) -> ()
            n329 = local read "`()` count"() -> (w574:u16)
            n330 = Increment(x=w574) -> (x+1=w573:u16)
            n331 = local write "`()` count"(w573) -> ()
          }
          frame 12 {
            # "check is \"(1/\""
            n332 = Reverse 1D Array(array=w595) -> (reversed array=w594:cluster{"op":u16, "number":dbl}[])
            n333 = for {
              tunnel: w594 -> [w614] mode=indexing
              shift-right: [w613] -> w591
              shift-left: _ -> [_]
              shift-right: [w609] -> _
              shift-left: 0 -> [w611]
              i -> [w613]
              stop <- w610 stop-if-true
              # "find correspond \"(\""
              n334 = Unbundle(w614) -> ("op"=w612:u16)  [unwired: 1 out]
              n335 = case shown="12" w612 {
                tunnel: [w615 w616 w618] -> w609
                tunnel: w611 -> [w615 w617 w619]
                frame 0, Default {
                }
                frame 11 {
                  n336 = Decrement(x=w617) -> (x-1=w616:i32)
                }
                frame 12 {
                  n337 = Increment(x=w619) -> (x+1=w618:i32)
                }
              }
              n338 = Equal To 0?(x=w609) -> (x = 0?=w610:bool)
            }
            n339 = Subtract(x=w592, y=w591) -> (x-y=w578:i32)
            n340 = Increment(x=w578) -> (x+1=w587:i32)
            n341 = Increment(x=w587) -> (x+1=w588:i32)
            n342 = Index Array(array=w579, index=w587) -> (element=w590:cluster{"op":u16, "number":dbl})
            n343 = Index Array(array=w579, index=w588) -> (element=w589:cluster{"op":u16, "number":dbl})
            n344 = Unbundle(w590) -> ("number"=w586:dbl)  [unwired: 1 out]
            n345 = Unbundle(w589) -> ("op"=w584:u16)  [unwired: 1 out]
            n346 = Equal?(x=w586, y=1.0) -> (x = y?=w581:bool)
            n347 = Equal?(x=w584, y=u16 6) -> (x = y?=w582:bool)
            n348 = And(x=w581, y=w582) -> (x .and. y?=w580:bool)
            n349 = case shown="False" w580 {
              tunnel: w579 -> [w603 w608]
              tunnel: w578 -> [w602 w606]
              tunnel: [w596 w604] -> w577
              frame False {
                n350 = Insert Into Array(array=w603, index=w602, new element #1=cluster{u16, dbl} {11, 0.0}, new element #2=cluster{u16, dbl} {1, 1.0}, new element #3=cluster{u16, dbl} {6, 0.0}) -> (w598:cluster{"op":u16, "number":dbl}[])
                n351 = Build Array (concatenate)(w598, cluster{u16, dbl} {12, 0.0}) -> (w596:cluster{"op":u16, "number":dbl}[])
              }
              frame True {
                n352 = Delete From Array(array=w608, length=3, index=w606) -> (array with subset deleted=w605:cluster{"op":u16, "number":dbl}[])  [unwired: 1 out]
                n353 = Delete From Array(array=w605) -> (array with subset deleted=w604:cluster{"op":u16, "number":dbl}[])  [unwired: 2 in, 1 out]
              }
            }
            n354 = local write "input queue"(w577) -> ()
          }
        }
      }
      frame 10 {
        # "check nagtive & start pos"
        n355 = local read "input queue"() -> (w621:cluster{"op":u16, "number":dbl}[])
        n356 = Array Size(array=w621) -> (size(s)=w623:i32)
        n357 = Decrement(x=w623) -> (x-1=w622:i32)
        n358 = Index Array(array=w621, index=w622) -> (element=w625:cluster{"op":u16, "number":dbl})
        n359 = Unbundle(w625) -> ("op"=w624:u16)  [unwired: 1 out]
        n360 = case shown="1, 2" w624 {
          tunnel: w621 -> [_ w629 w676 w683]
          tunnel: w622 -> [_ w633 _ _]
          tunnel: w620 -> [_ _ w671 w677]
          frame 7, Default {
            n361 = One Button Dialog(message="You can't place nagtive here!") -> ()  [unwired: 1 in, 1 out]
          }
          frame 1, 2 {
            n362 = Reverse 1D Array(array=w629) -> (reversed array=w634:cluster{"op":u16, "number":dbl}[])
            n363 = for {
              tunnel: w634 -> [w667] mode=indexing
              shift-right: [w665] -> w631
              shift-left: _ -> [_]
              i -> [w666]
              stop <- w659 stop-if-true
              n364 = Unbundle(w667) -> ("op"=w663:u16)  [unwired: 1 out]
              n365 = Not Equal?(x=w663, y=u16 1) -> (x != y?=w661:bool)
              n366 = Not Equal?(x=w663, y=u16 2) -> (x != y?=w660:bool)
              n367 = And(x=w661, y=w660) -> (x .and. y?=w659:bool)
              n368 = case shown="False" w659 {
                tunnel: w666 -> [w669 w670]
                tunnel: [w668 w670] -> w665
                frame False {
                  n369 = Increment(x=w669) -> (x+1=w668:i32)
                }
                frame True {
                }
              }
            }
            n370 = Subtract(x=w633, y=w631) -> (x-y=w630:i32)
            n371 = Index Array(array=w629, index=w630) -> (element=w628:cluster{"op":u16, "number":dbl})
            n372 = Unbundle(w628) -> ("op"=w627:u16)  [unwired: 1 out]
            n373 = case shown="5, 6" w627 {
              tunnel: [w637 w638 w642 w646 w651 w657] -> w632
              tunnel: w630 -> [_ w640 w644 w650 w653 w655]
              tunnel: w629 -> [w635 w641 w645 w649 w652 w658]
              frame 0 {
                n374 = Build Array (concatenate)(cluster{u16, dbl} {10, 0.0}, w635) -> (w637:cluster{"op":u16, "number":dbl}[])
              }
              frame 3 {
                n375 = Replace Array Subset(array=w641, new element=cluster{u16, dbl} {4, 0.0}, index=w640) -> (w638:cluster{"op":u16, "number":dbl}[])
              }
              frame 4 {
                n376 = Replace Array Subset(array=w645, new element=cluster{u16, dbl} {3, 0.0}, index=w644) -> (w642:cluster{"op":u16, "number":dbl}[])
              }
              frame 5, 6 {
                n377 = Increment(x=w650) -> (x+1=w647:i32)
                n378 = Insert Into Array(array=w649, index=w647, new element=cluster{u16, dbl} {10, 0.0}) -> (w646:cluster{"op":u16, "number":dbl}[])
              }
              frame 10 {
                n379 = Delete From Array(array=w652, index=w653) -> (array with subset deleted=w651:cluster{"op":u16, "number":dbl}[])  [unwired: 1 in, 1 out]
              }
              frame 11, Default {
                n380 = Increment(x=w655) -> (x+1=w654:i32)
                n381 = Insert Into Array(array=w658, index=w654, new element=cluster{u16, dbl} {10, 0.0}) -> (w657:cluster{"op":u16, "number":dbl}[])
              }
            }
            n382 = local write "input queue"(w632) -> ()
          }
          frame 0, 3..6, 11 {
            n383 = Build Array (concatenate)(w676, w671, cluster{u16, dbl} {11, 0.0}) -> (w674:cluster{"op":u16, "number":dbl}[])
            n384 = local write "input queue"(w674) -> ()
            n385 = local read "`()` count"() -> (w673:u16)
            n386 = Increment(x=w673) -> (x+1=w672:u16)
            n387 = local write "`()` count"(w672) -> ()
          }
          frame 12 {
            n388 = Build Array (concatenate)(w683, cluster{u16, dbl} {5, 0.0}, w677, cluster{u16, dbl} {11, 0.0}) -> (w682:cluster{"op":u16, "number":dbl}[])
            n389 = local read "`()` count"() -> (w679:u16)
            n390 = local write "input queue"(w682) -> ()
            n391 = Increment(x=w679) -> (x+1=w678:u16)
            n392 = local write "`()` count"(w678) -> ()
          }
        }
      }
      frame 11 {
        n393 = local read "input queue"() -> (w686:cluster{"op":u16, "number":dbl}[])
        n394 = Array Size(array=w686) -> (size(s)=w692:i32)
        n395 = Decrement(x=w692) -> (x-1=w691:i32)
        n396 = Index Array(array=w686, index=w691) -> (element=w690:cluster{"op":u16, "number":dbl})
        n397 = local read "`()` count"() -> (w694:u16)
        n398 = Unbundle(w690) -> ("op"=w689:u16)  [unwired: 1 out]
        n399 = Equal?(x=w689, y=u16 1) -> (x = y?=w687:bool)
        n400 = Increment(x=w694) -> (x+1=w693:u16)
        n401 = case shown="True" w687 {
          tunnel: w686 -> [w697 w701]
          tunnel: w685 -> [w696 w699]
          tunnel: [w695 w698] -> w684
          frame False {
            n402 = Build Array (concatenate)(w697, w696) -> (w695:cluster{"op":u16, "number":dbl}[])
          }
          frame True {
            n403 = Build Array (concatenate)(w701, cluster{u16, dbl} {5, 0.0}, w699) -> (w698:cluster{"op":u16, "number":dbl}[])
          }
        }
        n404 = local write "`()` count"(w693) -> ()
        n405 = local write "input queue"(w684) -> ()
      }
      frame 12 {
        n406 = local read "input queue"() -> (w703:cluster{"op":u16, "number":dbl}[])
        n407 = Array Size(array=w703) -> (size(s)=w712:i32)
        n408 = Decrement(x=w712) -> (x-1=w711:i32)
        n409 = local read "`()` count"() -> (w704:u16)
        n410 = Index Array(array=w703, index=w711) -> (element=w710:cluster{"op":u16, "number":dbl})
        n411 = Unbundle(w710) -> ("op"=w709:u16)  [unwired: 1 out]
        n412 = Less Or Equal To 0?(x=w704) -> (x <= 0?=w706:bool)
        n413 = Equal?(x=w709, y=u16 11) -> (x = y?=w707:bool)
        n414 = Or(x=w706, y=w707) -> (x .or. y?=w705:bool)
        n415 = case shown="True" w705 {
          tunnel: w704 -> [w717 _]
          tunnel: w703 -> [w714 _]
          tunnel: w702 -> [w713 _]
          frame False {
            n416 = Decrement(x=w717) -> (x-1=w716:u16)
            n417 = local write "`()` count"(w716) -> ()
            n418 = Build Array (concatenate)(w714, w713) -> (w715:cluster{"op":u16, "number":dbl}[])
            n419 = local write "input queue"(w715) -> ()
          }
          frame True {
            n420 = One Button Dialog(message="You can't place parentheses here!") -> ()  [unwired: 1 in, 1 out]
          }
        }
      }
      frame 20 {
        # "reset all input"
        n421 = Two Button Dialog(message="Confirm clear?", 1:"Cancel" ("F button name (\"Cancel\")"), 2:"Yes" ("T button name (\"OK\")")) -> (T button?=w719:bool)
        n422 = case shown="True" w719 {
          frame False {
          }
          frame True {
            n423 = xnode "Error Ring"() -> ("error out"=w724:errorcluster)
            n424 = invoke on="input queue" class="Arr (strict)" method="Reinit To Default"(error in=w724) -> ()  [unwired: 2 in, 3 out]
            n425 = local write "`()` count"(u16 0 ("`()` count")) -> ()
          }
        }
      }
      frame 21 {
        n426 = local read "input queue"() -> (w727:cluster{"op":u16, "number":dbl}[])
        n427 = while {
          shift-right: [w739] -> w726
          shift-left: w727 -> [w742]
          i -> [w738]
          stop <- w730 stop-if-true
          # "delete until not number or dot"
          n428 = Delete From Array(array=w742) -> (deleted portion=w740:cluster{"op":u16, "number":dbl}, array with subset deleted=w737:cluster{"op":u16, "number":dbl}[])  [unwired: 2 in]
          n429 = Unbundle(w740) -> ("op"=w728:u16)  [unwired: 1 out]
          n430 = Not Equal To 0?(x=w738) -> (x != 0?=w729:bool)
          n431 = Array Size(array=w737) -> (size(s)=w736:i32)
          n432 = Not Equal?(x=w728, y=u16 1) -> (x != y?=w732:bool)
          n433 = Not Equal?(x=w728, y=u16 2) -> (x != y?=w731:bool)
          n434 = Not Equal To 0?(x=w736) -> (x != 0?=w735:bool)
          n435 = And(x=w732, y=w731) -> (x .and. y?=w730:bool)
          n436 = Compound Arithmetic op=AND(w735, w730, w729) -> (w734:bool)
          n437 = case shown="False" w734 {
            tunnel: w740 -> [_ w761]
            tunnel: w737 -> [w743 w763]
            tunnel: [w744 w762] -> w739
            tunnel: w728 -> [w745 _]
            frame False {
              n438 = case shown="11" w745 {
                tunnel: w745 -> [_ _ _]
                tunnel: w743 -> [w746 w748 w758]
                tunnel: [w746 w747 w758] -> w744
                frame 0, Default {
                }
                frame 11 {
                  # "if ( with sqrt, delete it"
                  n439 = local read "`()` count"() -> (w754:u16)
                  n440 = Decrement(x=w754) -> (x-1=w753:u16)
                  n441 = local write "`()` count"(w753) -> ()
                  n442 = Array Size(array=w748) -> (size(s)=w749:i32)
                  n443 = Decrement(x=w749) -> (x-1=w750:i32)
                  n444 = Index Array(array=w748, index=w750) -> (element=w751:cluster{"op":u16, "number":dbl})
                  n445 = Unbundle(w751) -> ("op"=w752:u16)  [unwired: 1 out]
                  n446 = case shown="7, 10" w752 {
                    tunnel: w748 -> [w755 w757]
                    tunnel: [w755 w756] -> w747
                    frame 0, Default {
                    }
                    frame 7, 10 {
                      n447 = Delete From Array(array=w757) -> (array with subset deleted=w756:cluster{"op":u16, "number":dbl}[])  [unwired: 2 in, 1 out]
                    }
                  }
                }
                frame 12 {
                  n448 = local read "`()` count"() -> (w760:u16)
                  n449 = Increment(x=w760) -> (x+1=w759:u16)
                  n450 = local write "`()` count"(w759) -> ()
                }
              }
            }
            frame True {
              n451 = Build Array (concatenate)(w763, w761) -> (w762:cluster{"op":u16, "number":dbl}[])
            }
          }
        }
        n452 = local write "input queue"(w726) -> ()
      }
      frame 22 {
        # "remove last element"
        n453 = local read "input queue"() -> (w767:cluster{"op":u16, "number":dbl}[])
        n454 = Delete From Array(array=w767) -> (deleted portion=w765:cluster{"op":u16, "number":dbl}, array with subset deleted=w766:cluster{"op":u16, "number":dbl}[])  [unwired: 2 in]
        n455 = Unbundle(w765) -> ("op"=w764:u16)  [unwired: 1 out]
        n456 = local write "input queue"(w766) -> ()
        n457 = case shown="11" w764 {
          frame 0, Default {
          }
          frame 11 {
            n458 = local read "`()` count"() -> (w774:u16)
            n459 = Decrement(x=w774) -> (x-1=w773:u16)
            n460 = local write "`()` count"(w773) -> ()
            n461 = local read "input queue"() -> (w768:cluster{"op":u16, "number":dbl}[])
            n462 = Array Size(array=w768) -> (size(s)=w772:i32)
            n463 = Decrement(x=w772) -> (x-1=w771:i32)
            n464 = Index Array(array=w768, index=w771) -> (element=w770:cluster{"op":u16, "number":dbl})
            n465 = Unbundle(w770) -> ("op"=w769:u16)  [unwired: 1 out]
            n466 = case shown="7, 10" w769 {
              tunnel: w768 -> [_ w776]
              frame 0, Default {
              }
              frame 7, 10 {
                n467 = Delete From Array(array=w776) -> (array with subset deleted=w775:cluster{"op":u16, "number":dbl}[])  [unwired: 2 in, 1 out]
                n468 = local write "input queue"(w775) -> ()
              }
            }
          }
          frame 12 {
            n469 = local read "`()` count"() -> (w778:u16)
            n470 = Increment(x=w778) -> (x+1=w777:u16)
            n471 = local write "`()` count"(w777) -> ()
          }
        }
      }
    }
    n472 = for {
      shift-right: [w419] -> w41
      shift-left: "" -> [w420]
      tunnel: w40 -> [w424] mode=indexing
      n473 = Unbundle(w424) -> ("op"=w423:u16, "number"=w422:dbl)
      n474 = case shown="23" w423 {
        tunnel: w422 -> [_ w427 _ _ _ _ _ _ _ _ _ _]
        tunnel: ["" w426 "." "+" "-" "×" "÷" "√" "-" "(" ")" w439] -> w421
        frame 0, Default {
        }
        frame 1 {
          n475 = Number To Decimal String(number=w427) -> (decimal integer string=w426:string)  [unwired: 1 in]
        }
        frame 2 {
        }
        frame 3 {
        }
        frame 4 {
        }
        frame 5 {
        }
        frame 6 {
        }
        frame 7 {
        }
        frame 10 {
          # "negtive"
        }
        frame 11 {
        }
        frame 12 {
        }
        frame 23 {
          n476 = local read "result str"() -> (w438:string)
          n477 = Concatenate Strings("=", "\r", w438) -> (w439:string)
        }
      }
      n478 = Concatenate Strings(w420, w421) -> (w419:string)
    }
    "screen" <- w41
  }
